vi "Host_Main.vi"() -> ()   [LabVIEW 2018]
doc: "Use this template to build a VI to use as a subVI."
panel:
  out "Exit Error":errorcluster
  out "MES Error":errorcluster
  out "Upload Code":string
  out "Pending Count":i32
  out "Upload OK":bool
  out "Exit Status":string
  in  "Test Exit":bool
  in  "Exit":bool
  in  "Bin Cap":u16=20
  in  "Timeout":u16=50
  in  "Speed %":u16=60
  in  "Clear Bin":bool
  in  "Bin Full":bool
  in  "Clamp Stuck":bool
  in  "E-Stop":bool
  in  "Reset":bool
  in  "Cycle Stop":bool
  in  "Test Start":bool
  in  "Start":bool
  out "NG Bin":u16
  out "Total":u16
  out "NG Count":u16
  out "OK Count":u16
  out "SafetyOK":bool
  out "Stop Req":bool
  out "Alarm":bool
  out "Alarm Code":u16
  out "Alarm Text":string
  out "Step":string
  out "PLC Connected":bool
  out "Line Picture":picture
  out "Servo Error":errorcluster
  out "Inspect Error":errorcluster
  in  "Log Dir":path=path "D:/aoi_log"
  out "Surface Defect":string
  out "Width Defect":string
  out "Pins Defect":string
  out "Surface OK":bool
  out "Width OK":bool
  out "Pins OK":bool
  out "Part OK":bool
  in  "COM Port":refnum<visa-resource-name>
  in  "PLC Port":u16=5551
  in  "PLC Host":string="127.0.0.1"
  in  "PLC Transport":enum16{"TCP", "COM"}(ring)
  in  "Pause Heartbeat":bool
  out "Init Error":errorcluster
  out "Lot Code":string
  out "Lot Started":bool
  in  "Lot No":string="L2610-001"
  in  "Recipe Name":string="CN-08"
  in  "Recipe Dir":path
  # "SETUP"
  # "STATUS"
  # "OPERATION"
  # "INSPECTION"
  # "TRAINING"
  # "ALARM TABLE"
  # "MES"
  # "8001  ESTOP                 8004  AIR LOW\n8101  NG BIN FULL\n9001  STOPPER TIMEOUT\n9002  CLAMP TIMEOUT\n9003  PUSHER TIMEOUT\n9004  PART NOT ARRIVED\n9005  INSPECT TIMEOUT\n9006  HEARTBEAT TIMEOUT\n9007  BAD RESULT\n9008  SERVO ALARM"
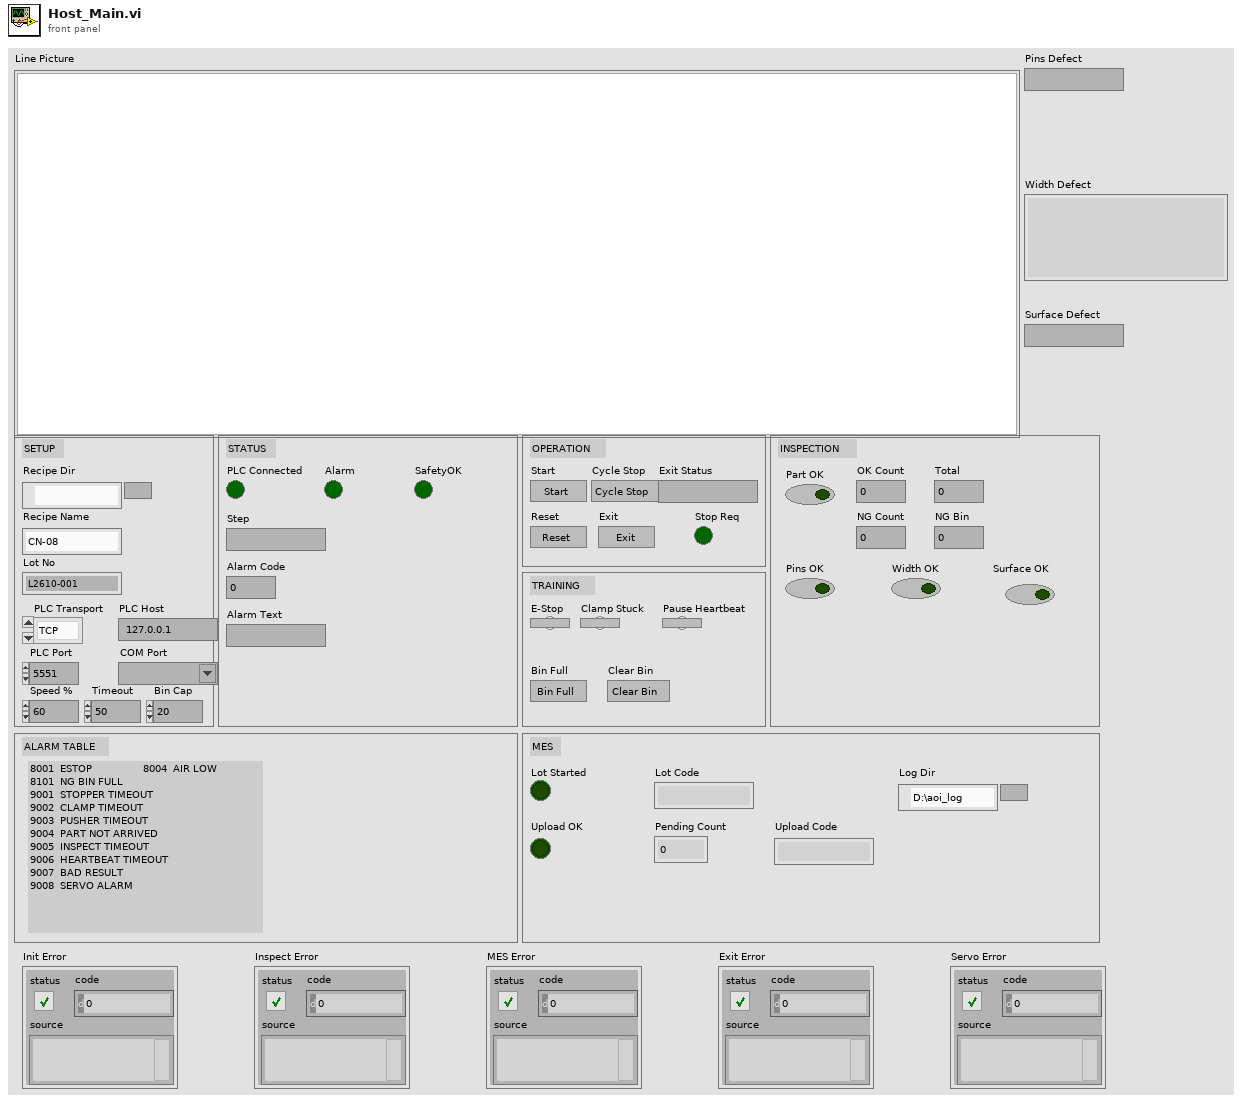
[diagram p1: front panel]
types:
  T1 = typedef "Recipe.ctl" = cluster{"recipe":string, "pins_x_mm":dbl, "pins_count":i32, "pins_pitch_mm":dbl, "width_x_mm":dbl, "width_nominal_mm":dbl, "surface_max_dark_px":i32, "surface_dark_level":dbl, "surface_x_mm":dbl, "width_tol_mm":dbl, "pins_pitch_tol_mm":dbl}
  T2 = typedef "LV_Snapshot.ctl" = cluster{"DI":bool[], "DO":bool[], "IR":u16[], "Speed":u16}
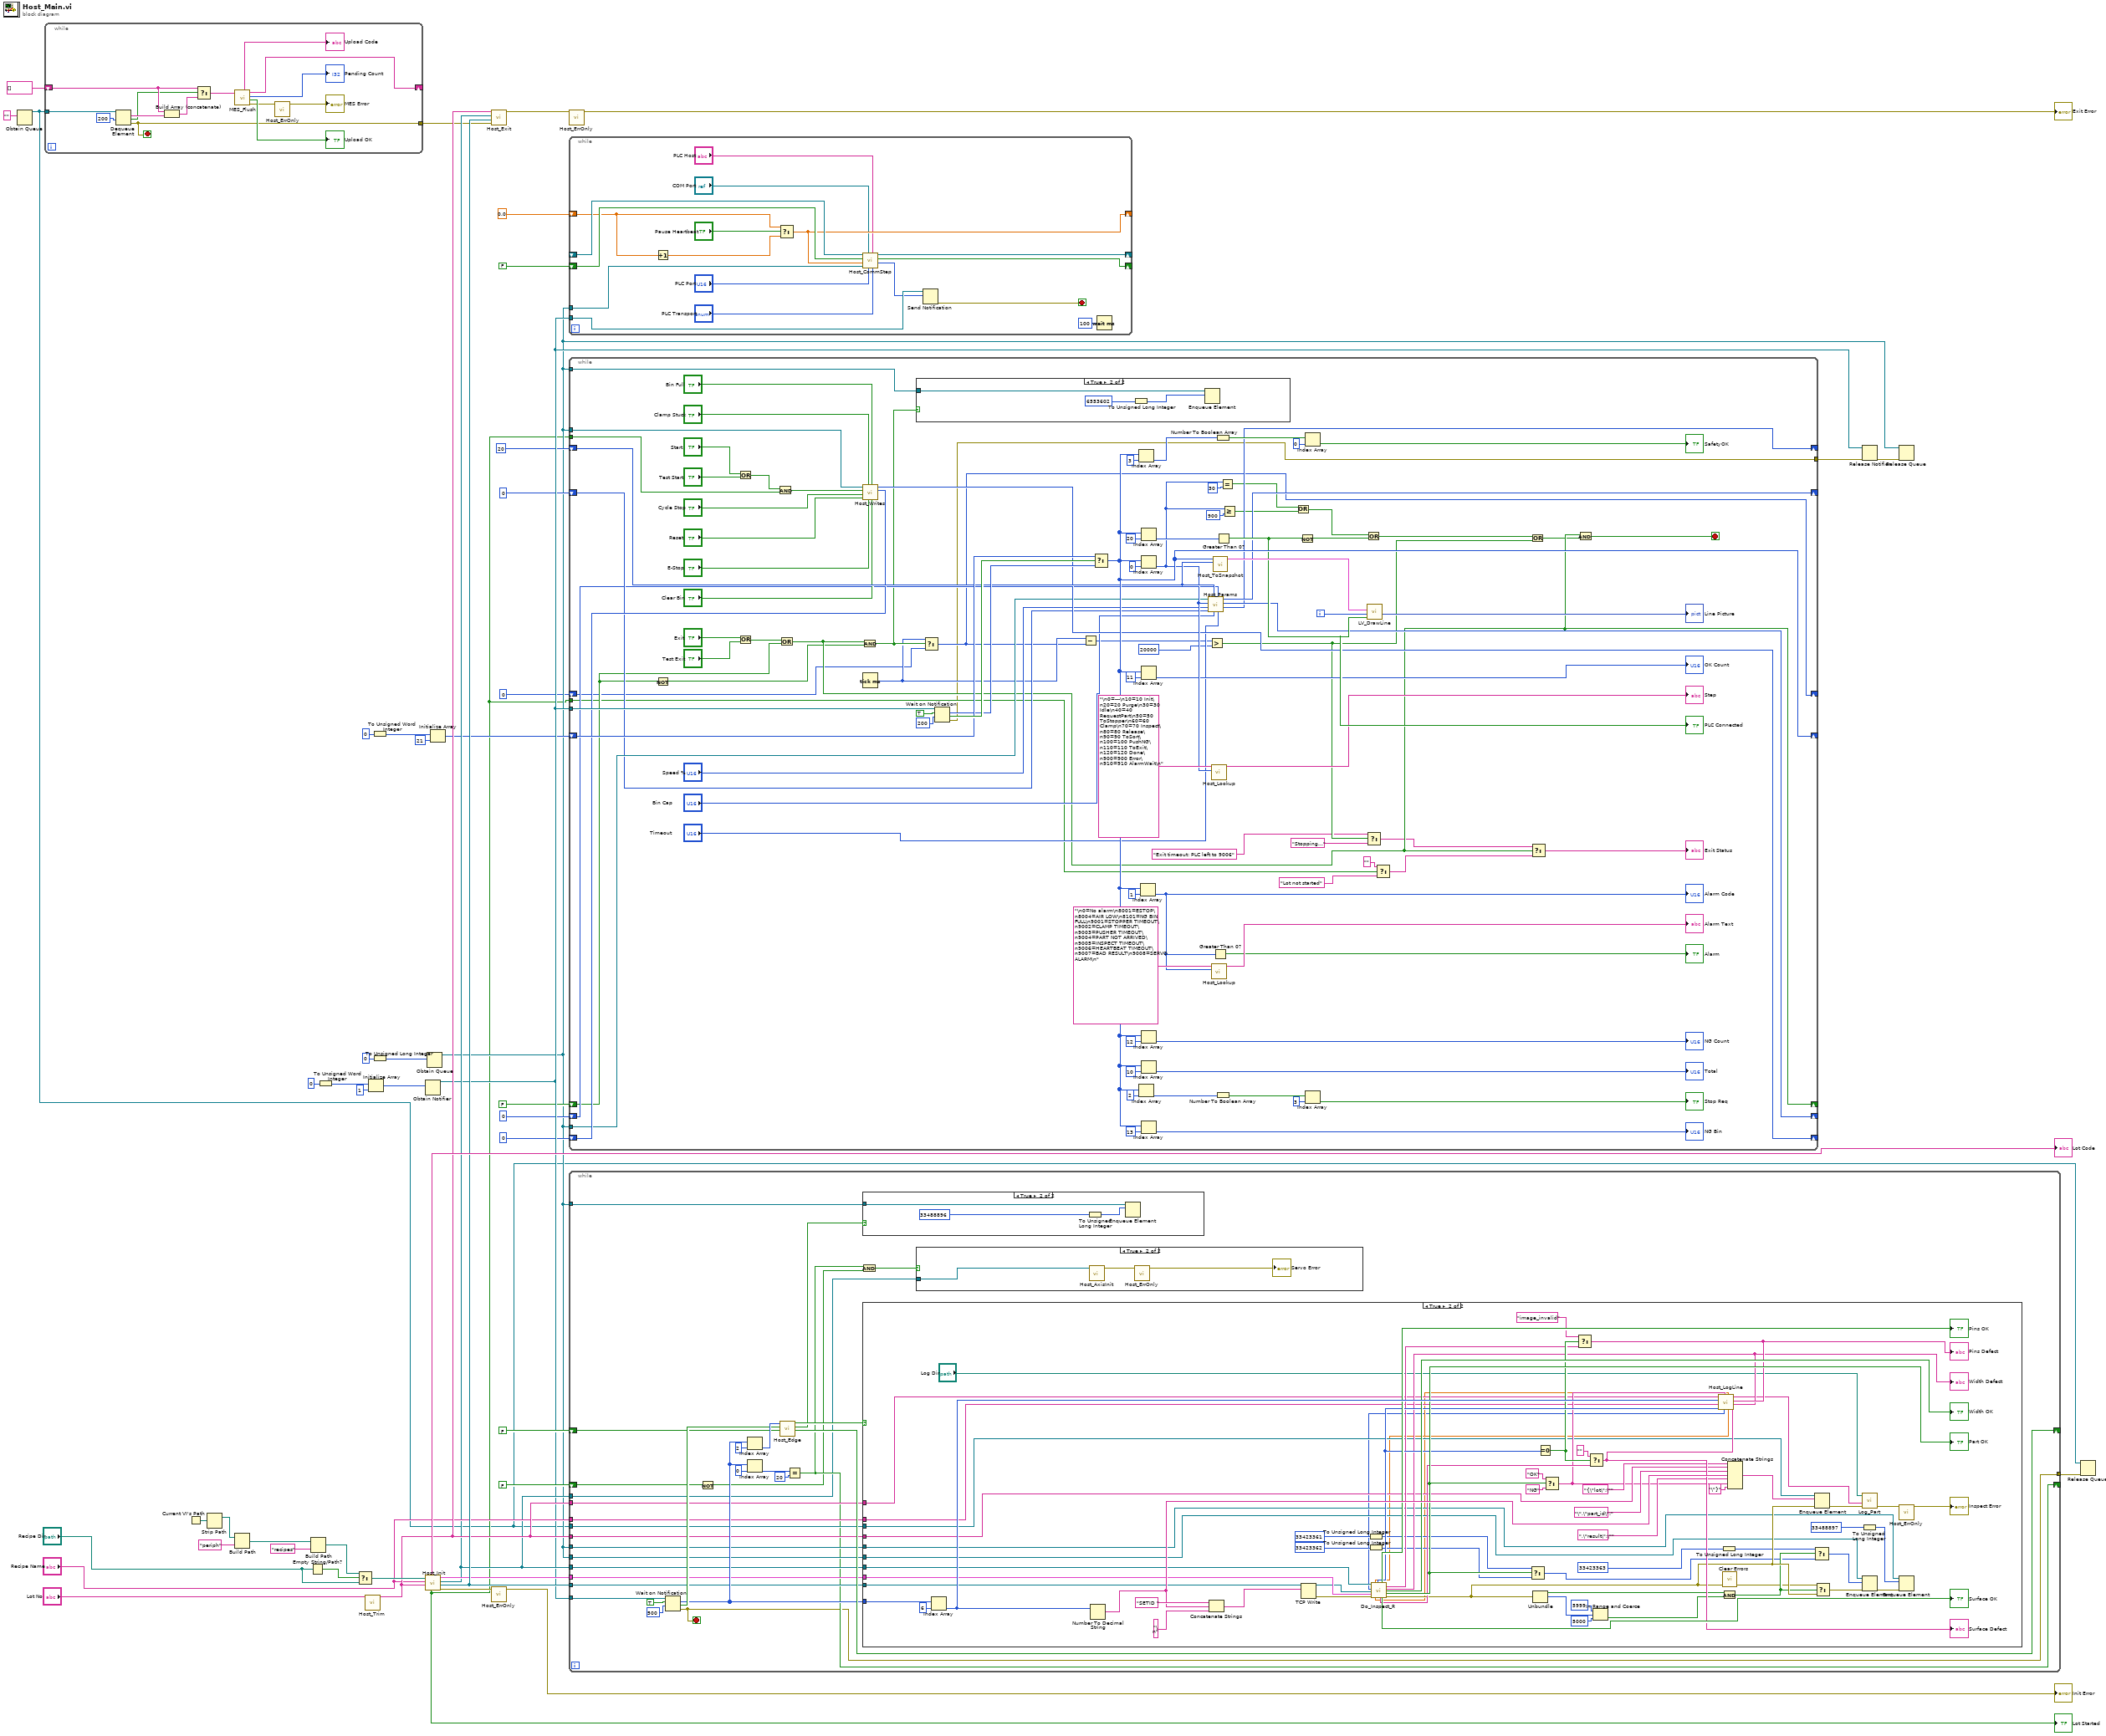
[diagram p0: block diagram]
diagram:
  n1 = Obtain Queue(element data type="") -> (queue out=w8:refnum<queue>)  [unwired: 4 in, 2 out]
  n2 = while {
    shift-right: [w57] -> _
    shift-left: string[] [] ("Pending in") -> [w62]
    tunnel: w8 -> [w64]
    tunnel: [w51] -> w3
    stop <- w51 stop-if-true
    n3 = Dequeue Element(queue=w64, timeout in ms (-1)=200) -> (element=w61:string, timed out?=w60:bool, error out=w51:errorcluster)  [unwired: 1 in, 1 out]
    n4 = Build Array (concatenate)(w62, w61) -> (w59:string[])
    n5 = Select(t=w62, s=w60, f=w59) -> (s? t:f=w58:string[])
    n6 = call "MES_Flush.vi"("Pending in"=w58) -> ("MES Error"=w53:errorcluster, "Upload OK"=→"Upload OK":bool, "Pending Count"=→"Pending Count":i32, "Pending out"=w57:string[], "Upload Code"=→"Upload Code":string)  [unwired: 6 in]
    n7 = call "Host_ErrOnly.vi"("error in"=w53) -> ("error out"=→"MES Error":errorcluster)  [unwired: 10 in]
  }
  n8 = Current VI's Path() -> (path=w43:path)
  n9 = Strip Path(path=w43) -> (stripped path=w42:path)  [unwired: 1 out]
  n10 = Build Path(base path=w42, name or relative path="periph") -> (appended path=w40:path)
  n11 = Empty String/Path?(string/path="Recipe Dir") -> (empty?=w37:bool)
  n12 = Build Path(base path=w40, name or relative path="recipes") -> (appended path=w36:path)
  n13 = To Unsigned Word Integer(number=0) -> (unsigned 16bit integer=w45:u16)
  n14 = Select(t=w36, s=w37, f="Recipe Dir") -> (s? t:f=w35:path)
  n15 = call "Host_Trim.vi"("string"="Lot No") -> ("trimmed string"=w25:string)  [unwired: 10 in]
  n16 = Initialize Array(w45, 1 ("dimension size")) -> (w44:u16[])
  n17 = To Unsigned Word Integer(number=0) -> (unsigned 16bit integer=w18:u16)
  n18 = To Unsigned Long Integer(number=0) -> (unsigned 32bit integer=w49:u32)
  n19 = Obtain Notifier(notification data type=w44) -> (notifier out=w21:refnum<notifier>)  [unwired: 3 in, 2 out]
  n20 = call "Host_Init.vi"("Lot No"=w25, "Recipe Name"="Recipe Name", "Recipe Dir"=w35) -> ("error out"=w32:errorcluster, "Camera"=w27:refnum<k5>, "Motion"=w22:refnum<visa-resource-name>, "Recipe"=w26:T1, "MES OK"=w9:bool, "MES Code"=→"Lot Code":string)  [unwired: 3 in]
  "Lot Started" <- w9
  n21 = Obtain Queue(element data type=w49) -> (queue out=w11:refnum<queue>)  [unwired: 4 in, 2 out]
  n22 = Initialize Array(w18, 21 ("dimension size")) -> (w17:u16[])
  n23 = call "Host_Exit.vi"("error in"=w3, "Camera"=w27, "Motion"=w22, "Lot No"=w25) -> ("error out"=w2:errorcluster)  [unwired: 7 in]
  n24 = call "Host_ErrOnly.vi"("error in"=w32) -> ("error out"=→"Init Error":errorcluster)  [unwired: 10 in]
  n25 = call "Host_ErrOnly.vi"("error in"=w2) -> ("error out"=→"Exit Error":errorcluster)  [unwired: 10 in]
  n26 = while {
    shift-right: [w78] -> _
    shift-left: _ -> [w80]
    shift-right: [w77] -> _
    shift-left: FALSE -> [w79]
    shift-right: [w73] -> _
    shift-left: 0.0 -> [w76]
    tunnel: w11 -> [w81]
    tunnel: w21 -> [w68]
    stop <- w65 stop-if-true
    n27 = Increment(x=w76) -> (x+1=w74:dbl)
    n28 = Select(t=w76, s="Pause Heartbeat", f=w74) -> (s? t:f=w73:dbl)
    n29 = call "Host_CommStep.vi"("Transport"="PLC Transport", "Host"="PLC Host", "Port"="PLC Port", "COM Port"="COM Port", "Queue"=w81, "Beat"=w73, "Connected"=w79, "PLC Conn"=w80) -> ("Words"=w67:u16[], "Connected out"=w77:bool, "PLC Conn out"=w78:refnum<visa-resource-name>)  [unwired: 1 in]
    n30 = Send Notification(notification=w67, notifier=w68) -> (error out=w65:errorcluster)  [unwired: 1 in, 1 out]
    n31 = Wait (ms)(milliseconds to wait=u32 100) -> ()  [unwired: 1 out]
  }
  n32 = while {
    shift-right: [w171] -> _
    shift-left: w17 -> [w173]
    shift-right: [w134] -> _
    shift-left: u16 0 ("Fault") -> [w135]
    shift-right: [w109] -> _
    shift-left: FALSE -> [w110]
    shift-right: [w103] -> _
    shift-left: u32 0 ("millisecond timer value") -> [w104]
    shift-right: [w119] -> _
    shift-left: u16 0 ("Next Speed") -> [w120]
    shift-right: [w116] -> _
    shift-left: u16 0 ("Next Timeout") -> [w117]
    shift-right: [w114] -> _
    shift-left: u16 20 ("Next Capacity") -> [w170]
    tunnel: w21 -> [w177]
    tunnel: w11 -> [w136]
    tunnel: w9 -> [w130]
    tunnel: w11 -> [w122]
    tunnel: w11 -> [w106]
    tunnel: w9 -> [w87]
    tunnel: [w82] -> w6
    i -> [w165]
    stop <- w91 stop-if-true
    n33 = Not(x=w110) -> (.not. x?=w108:bool)
    n34 = Or(x="Start", y="Test Start") -> (x .or. y?=w131:bool)
    n35 = Or(x="Exit", y="Test Exit") -> (x .or. y?=w111:bool)
    n36 = And(x=w131, y=w130) -> (x .and. y?=w129:bool)
    n37 = Or(x=w111, y=w110) -> (x .or. y?=w109:bool)
    n38 = call "Host_Writes.vi"("Prev Fault"=w135, "Clear Bin"="Clear Bin", "Bin Full"="Bin Full", "E-Stop"="E-Stop", "Clamp Stuck"="Clamp Stuck", "Reset"="Reset", "Stop"="Cycle Stop", "Start"=w129, "Queue"=w136) -> ("Fault"=w134:u16)  [unwired: 2 in]
    n39 = And(x=w109, y=w108) -> (x .and. y?=w107:bool)
    n40 = Tick Count (ms)() -> (millisecond timer value=w105:u32)
    n41 = case shown="True" w107 {
      tunnel: w106 -> [_ w179]
      frame False {
      }
      frame True {
        n42 = To Unsigned Long Integer(number=6553602) -> (unsigned 32bit integer=w178:u32)
        n43 = Enqueue Element(queue=w179, element=w178) -> ()  [unwired: 2 in, 3 out]
      }
    }
    n44 = Select(t=w105, s=w107, f=w104) -> (s? t:f=w103:u32)
    n45 = Wait on Notification(notifier=w177, ignore previous (F)=TRUE, timeout in ms (-1)=200) -> (notification=w172:u16[], timed out?=w174:bool, error out=w82:errorcluster)  [unwired: 1 in, 1 out]
    n46 = Subtract(x=w105, y=w103) -> (x-y=w102:u32)
    n47 = Select(t=w173, s=w174, f=w172) -> (s? t:f=w171:u16[])
    n48 = Index Array(array=w171, index=3) -> (element=w148:u16)
    n49 = Index Array(array=w171, index=2) -> (element=w153:u16)
    n50 = Index Array(array=w171, index=1) -> (element=w157:u16)
    "Alarm Code" <- w157
    n51 = Index Array(array=w171, index=20) -> (element=w168:u16)
    n52 = Index Array(array=w171, index=0) -> (element=w160:u16)
    n53 = Index Array(array=w171, index=11) -> (element=→"OK Count":u16)
    n54 = Index Array(array=w171, index=12) -> (element=→"NG Count":u16)
    n55 = Index Array(array=w171, index=10) -> (element=→"Total":u16)
    n56 = Index Array(array=w171, index=13) -> (element=→"NG Bin":u16)
    n57 = call "Host_Params.vi"("Timeout"="Timeout", "Prev Timeout"=w117, "Capacity"="Bin Cap", "Prev Capacity"=w170, "Prev Speed"=w120, "Speed"="Speed %", "Step"=w160, "Queue"=w122) -> ("Next Capacity"=w114:u16, "Next Timeout"=w116:u16, "Next Speed"=w119:u16)  [unwired: 1 in]
    n58 = Greater?(x=w102, y=u32 20000) -> (0:w93:bool)
    n59 = call "Host_Lookup.vi"("Key"=w160, "Table"="\n0=---\n10=10 Init\n20=20 Purge\n30=30 Idle\n40=40 RequestPart\n50=50 ToStopper\n60=60 Clamp\n70=70 Inspect\n80=80 Release\n90=90 ToSort\n100=100 PushNG\n110=110 ToExit\n120=120 Done\n900=900 Error\n910=910 AlarmWait\n") -> ("Text"=→"Step":string)  [unwired: 9 in]
    n60 = call "Host_Lookup.vi"("Key"=w157, "Table"="\n0=No alarm\n8001=ESTOP\n8004=AIR LOW\n8101=NG BIN FULL\n9001=STOPPER TIMEOUT\n9002=CLAMP TIMEOUT\n9003=PUSHER TIMEOUT\n9004=PART NOT ARRIVED\n9005=INSPECT TIMEOUT\n9006=HEARTBEAT TIMEOUT\n9007=BAD RESULT\n9008=SERVO ALARM\n") -> ("Text"=→"Alarm Text":string)  [unwired: 9 in]
    n61 = call "Host_ToSnapshot.vi"("Bin Cap"=w170, "Words"=w171) -> ("Snapshot"=w167:T2)  [unwired: 9 in]
    n62 = Greater Than 0?(x=w157) -> (x > 0?=→"Alarm":bool)
    n63 = Number To Boolean Array(number=w148) -> (Boolean array=w147:bool[])
    n64 = Number To Boolean Array(number=w153) -> (Boolean array=w152:bool[])
    n65 = Greater Than 0?(x=w168) -> (x > 0?=w166:bool)
    "PLC Connected" <- w166
    n66 = Equal?(x=w160, y=u16 30) -> (x = y?=w98:bool)
    n67 = Greater Or Equal?(x=w160, y=u16 900) -> (x >= y?=w97:bool)
    n68 = Or(x=w98, y=w97) -> (x .or. y?=w96:bool)
    n69 = Not(x=w166) -> (.not. x?=w95:bool)
    n70 = Index Array(array=w147, index=0) -> (element=→"SafetyOK":bool)
    n71 = Index Array(array=w152, index=3) -> (element=→"Stop Req":bool)
    n72 = Or(x=w96, y=w95) -> (x .or. y?=w94:bool)
    n73 = Select(t="Exit timeout: PLC left to 9006", s=w93, f="Stopping...") -> (s? t:f=w88:string)
    n74 = call "LV_DrawLine.vi"("Connected"=w166, "Phase"=w165, "Snapshot"=w167) -> ("Line Picture"=→"Line Picture":picture)  [unwired: 8 in]
    n75 = Select(t="", s=w87, f="Lot not started") -> (s? t:f=w84:string)
    n76 = Or(x=w94, y=w93) -> (x .or. y?=w92:bool)
    n77 = Select(t=w88, s=w109, f=w84) -> (s? t:f=→"Exit Status":string)
    n78 = And(x=w109, y=w92) -> (x .and. y?=w91:bool)
  }
  n79 = while {
    shift-right: [w203] -> _
    shift-left: FALSE -> [w204]
    tunnel: w21 -> [w210]
    tunnel: w27 -> [w200]
    tunnel: w26 -> [w199]
    tunnel: w22 -> [w198]
    tunnel: w11 -> [w197]
    tunnel: w11 -> [w196]
    tunnel: w25 -> [w195]
    tunnel: w8 -> [w194]
    tunnel: w25 -> [w193]
    tunnel: "Recipe Name" -> [w192]
    tunnel: w11 -> [w190]
    shift-right: [w186] -> _
    shift-left: FALSE -> [w185]
    tunnel: w22 -> [w182]
    tunnel: [w181] -> w4
    stop <- w181 stop-if-true
    n80 = Wait on Notification(notifier=w210, ignore previous (F)=TRUE, timeout in ms (-1)=500) -> (notification=w201:u16[], timed out?=w205:bool, error out=w181:errorcluster)  [unwired: 1 in, 1 out]
    n81 = Not(x=w185) -> (.not. x?=w184:bool)
    n82 = Index Array(array=w201, index=2) -> (element=w206:u16)
    n83 = Index Array(array=w201, index=0) -> (element=w188:u16)
    n84 = call "Host_Edge.vi"("Prev"=w204, "Timed Out"=w205, "Status"=w206) -> ("Next"=w203:bool, "Falling"=w191:bool, "Rising"=w202:bool)  [unwired: 6 in]
    n85 = Equal?(x=w188, y=u16 20) -> (x = y?=w186:bool)
    n86 = And(x=w186, y=w184) -> (x .and. y?=w183:bool)
    n87 = case shown="True" w191 {
      tunnel: w190 -> [_ w215]
      frame False {
      }
      frame True {
        n88 = To Unsigned Long Integer(number=33488896) -> (unsigned 32bit integer=w214:u32)
        n89 = Enqueue Element(queue=w215, element=w214) -> ()  [unwired: 2 in, 3 out]
      }
    }
    n90 = case shown="True" w202 {
      tunnel: w201 -> [_ w283]
      tunnel: w200 -> [_ w277]
      tunnel: w199 -> [_ w275]
      tunnel: w198 -> [_ w274]
      tunnel: w197 -> [_ w243]
      tunnel: w196 -> [_ w239]
      tunnel: w195 -> [_ w233]
      tunnel: w194 -> [_ w228]
      tunnel: w193 -> [_ w226]
      tunnel: w192 -> [_ w225]
      frame False {
      }
      frame True {
        n91 = Index Array(array=w283, index=6) -> (element=w281:u16)
        n92 = Number To Decimal String(number=w281) -> (decimal integer string=w279:string)  [unwired: 1 in]
        n93 = Concatenate Strings("SETID ", w279, "\n") -> (w276:string)
        n94 = TCP Write(connection ID=w277, data in=w276) -> (connection ID out=w273:refnum<k5>, error out=w272:errorcluster)  [unwired: 2 in, 1 out]
        n95 = To Unsigned Long Integer(number=33423361) -> (unsigned 32bit integer=w257:u32)
        n96 = To Unsigned Long Integer(number=33423362) -> (unsigned 32bit integer=w255:u32)
        n97 = call "Do_Inspect_R.vi"("VISA Refnum in"=w274, "connection ID"=w273, "Recipe"=w275, "error in (no error)"=w272) -> ("Dark Pixels"=w222:i16, "Pitch (mm)"=w224:dbl[], "Width (mm)"=w223:dbl, "Pin Count"=w267:i32, "Surface Defect"=w262:string, "Pins OK"=→"Pins OK":bool, "Surface OK"=→"Surface OK":bool, "Defect"=w264:string, "Width Defect"=w260:string, "Width OK"=→"Width OK":bool, "Part OK"=w271:bool, "error out"=w254:errorcluster)  [unwired: 1 in, 3 out]
        "Part OK" <- w271
        "Width Defect" <- w260
        n98 = Select(t=w257, s=w271, f=w255) -> (s? t:f=w244:u32)
        n99 = Unbundle(w254) -> ("status"=w250:bool, "code"=w253:i32)  [unwired: 1 out]
        n100 = Equal To 0?(x=w267) -> (x = 0?=w266:bool)
        n101 = Select(t="OK", s=w271, f="NG") -> (s? t:f=w230:string)
        n102 = Select(t="image_invalid", s=w266, f=w264) -> (s? t:f=w261:string)
        "Pins Defect" <- w261
        n103 = Select(t="", s=w266, f=w262) -> (s? t:f=w259:string)
        "Surface Defect" <- w259
        n104 = In Range and Coerce(upper limit=5999, x=w253, lower limit=5000) -> (In Range?=w249:bool)  [unwired: 1 out]
        n105 = call "Host_LogLine.vi"("Surface Defect"=w259, "Width Defect"=w260, "Defect"=w261, "Pitch (mm)"=w224, "Width (mm)"=w223, "Dark Pixels"=w222, "Result"=w230, "Pin Count"=w267, "Recipe Name"=w225, "Part ID"=w281, "Lot"=w226) -> ("Line"=w221:string)
        n106 = To Unsigned Long Integer(number=33423363) -> (unsigned 32bit integer=w245:u32)
        n107 = call <vilib>:"Clear Errors.vi"("error in (no error)"=w254) -> ("error out"=w247:errorcluster)  [unwired: 5 in, 1 out]
        n108 = And(x=w250, y=w249) -> (x .and. y?=w248:bool)
        n109 = Concatenate Strings("{\"lot\":\"", w233, "\",\"part_id\":", w279, ",\"result\":\"", w230, "\"}") -> (w227:string)
        n110 = Select(t=w245, s=w248, f=w244) -> (s? t:f=w242:u32)
        n111 = Enqueue Element(queue=w228, element=w227, error in (no error)=w254) -> (error out=w220:errorcluster)  [unwired: 1 in, 2 out]
        n112 = Select(t=w247, s=w248, f=w254) -> (s? t:f=w241:errorcluster)
        n113 = To Unsigned Long Integer(number=33488897) -> (unsigned 32bit integer=w238:u32)
        n114 = call "Log_Part.vi"("error in (no error)"=w220, "Line"=w221, "Log Dir"="Log Dir") -> ("error out"=w218:errorcluster)  [unwired: 8 in]
        n115 = Enqueue Element(queue=w243, element=w242, error in (no error)=w241) -> (error out=w237:errorcluster)  [unwired: 1 in, 2 out]
        n116 = call "Host_ErrOnly.vi"("error in"=w218) -> ("error out"=→"Inspect Error":errorcluster)  [unwired: 10 in]
        n117 = Enqueue Element(queue=w239, element=w238, error in (no error)=w237) -> ()  [unwired: 1 in, 3 out]
      }
    }
    n118 = case shown="True" w183 {
      tunnel: w182 -> [_ w213]
      frame False {
      }
      frame True {
        n119 = call "Host_AxisInit.vi"("Motion"=w213) -> ("error out"=w212:errorcluster)  [unwired: 10 in]
        n120 = call "Host_ErrOnly.vi"("error in"=w212) -> ("error out"=→"Servo Error":errorcluster)  [unwired: 10 in]
      }
    }
  }
  n121 = Release Notifier(notifier=w21, error in (no error)=w6) -> (error out=w5:errorcluster)  [unwired: 1 in, 2 out]
  n122 = Release Queue(queue=w11, error in (no error)=w5) -> ()  [unwired: 1 in, 3 out]
  n123 = Release Queue(queue=w8, error in (no error)=w4) -> ()  [unwired: 1 in, 3 out]
